vi "Set Name.vi"(8 "error in":errorcluster, 10 "Name":string, 11 "IElement in":refnum<class "IElement.lvclass">) -> (0 "error out":errorcluster, 3 "IElement out":refnum<class "IElement.lvclass">)   [LabVIEW 2026, in "IElement.lvclass"]
doc: "Set Name"
uses:
  IElement.lvclass
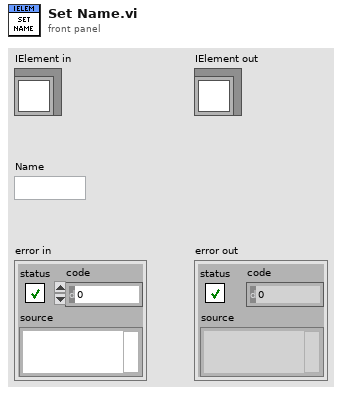
[diagram p1: front panel]
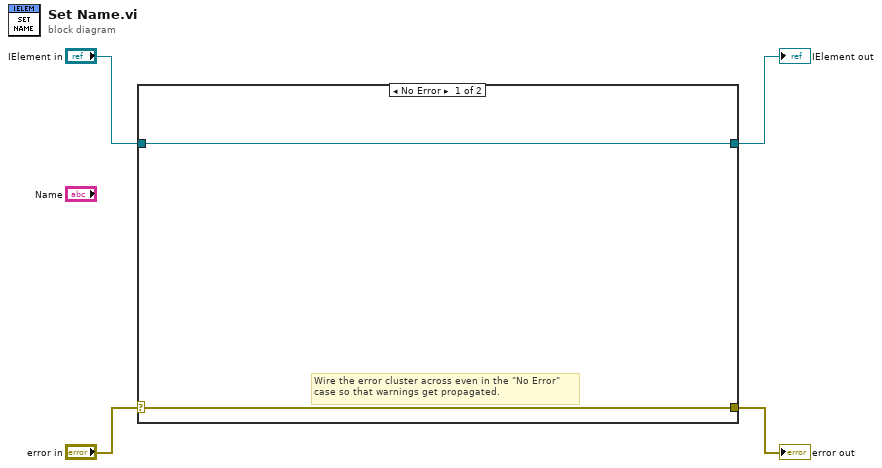
[diagram p0: block diagram]
diagram:
  n1 = case shown="No Error" "error in" {
    selector: "error in" -> [w6 w8]
    tunnel: [w6 w8] -> w3
    tunnel: [w5 w7] -> w1
    tunnel: "IElement in" -> [w5 w7]
    frame No Error {
      # "Wire the error cluster across even in the \"No Error\"\ncase so that warnings get propagated."
    }
    frame Error {
    }
  }
  "error out" <- w3
  "IElement out" <- w1
